vi "Send_TX.vi"(6 "frames (1)":u32=1, 7 "TLS connection":refnum<k5>, 8 "error in (no error)":errorcluster, 9 "status in":T1, 10 "length":i32, 11 "tx":u8[](array[numeric])) -> (0 "error out":errorcluster, 1 "status out":T1)   [LabVIEW 2021, in "CANsub_API.lvlib"]
doc: "API private: sends the first length bytes of the TX buffer with one TCP Write (1000 ms), counts frames written. TCP error ? state = Lost, error 5203. Loop-safe: no allocation, bounded time (except LabVIEW’s TCP Write string)."
uses:
  CANsub_API.lvlib
  Typedefs/CANsub_State.ctl
  common/Typedefs/Bit_Timing.ctl
  common/CANsub_Common.lvlib
  Typedefs/CANsub_Status.ctl
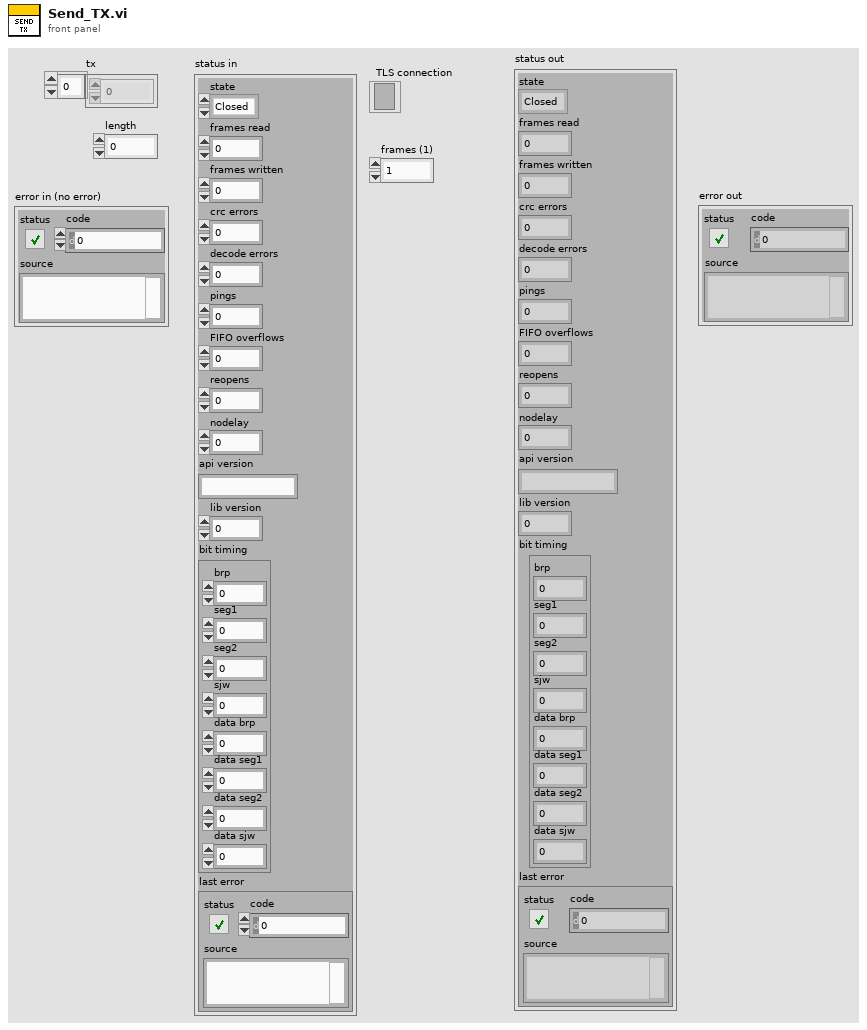
[diagram p1: front panel]
types:
  T1 = typedef "CANsub_API.lvlib/CANsub_Status.ctl" = cluster{"state":T2, "frames read":u32, "frames written":u32, "crc errors":u32, "decode errors":i32, "pings":u32, "FIFO overflows":u32, "reopens":u32, "nodelay":i32, "api version":string, "lib version":u32, "bit timing":T3, "last error":errorcluster}
  T2 = typedef "CANsub_API.lvlib/CANsub_State.ctl" = enum16{"Closed", "Open", "Lost"}
  T3 = typedef "CANsub_Common.lvlib/Bit_Timing.ctl" = cluster{"brp":u16, "seg1":u16, "seg2":u16, "sjw":u16, "data brp":u16, "data seg1":u16, "data seg2":u16, "data sjw":u16}
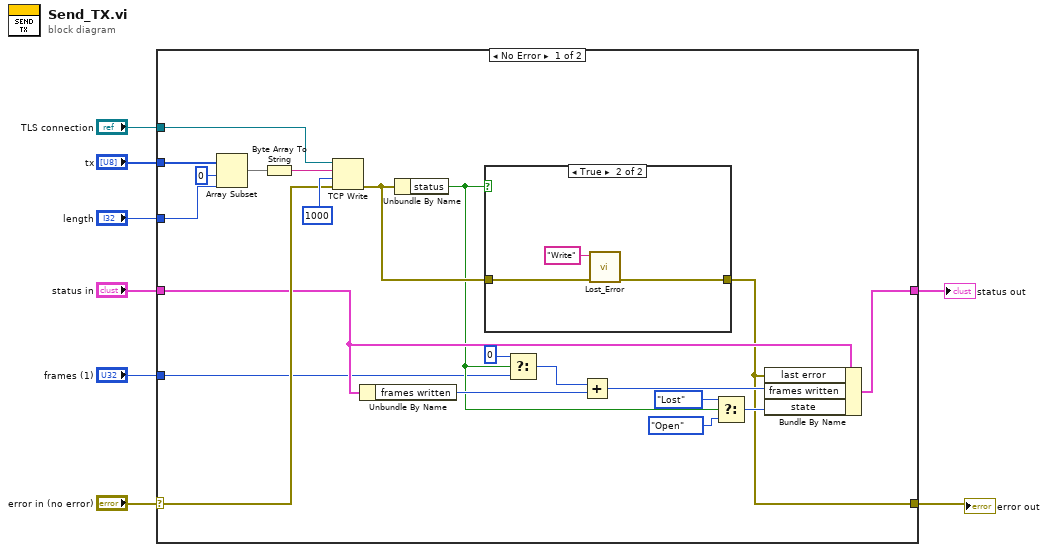
[diagram p0: block diagram]
diagram:
  n1 = case shown="No Error" "error in (no error)" {
    selector: "error in (no error)" -> [w22 w35]
    tunnel: [w10 w35] -> w7
    tunnel: [w19 w34] -> w6
    tunnel: "status in" -> [w20 w34]
    tunnel: "tx" -> [w29 _]
    tunnel: "length" -> [w28 _]
    tunnel: "TLS connection" -> [w24 _]
    tunnel: "frames (1)" -> [w9 _]
    frame No Error {
      n2 = Array Subset(array=w29, index=0, length=w28) -> (w26:u8[])
      n3 = Byte Array To String(unsigned byte array=w26) -> (string=w25:string)
      n4 = TCP Write(connection ID=w24, data in=w25, error in (no error)=w22, 9:1000 ("timeout ms (25000)")) -> (error out=w21:errorcluster)  [unwired: 2 out]
      n5 = Unbundle By Name(w20) -> ("frames written"=w18:u32)
      n6 = Unbundle By Name(w21) -> ("status"=w14:bool)
      n7 = case shown="True" w14 {
        tunnel: w21 -> [w30 w32]
        tunnel: [w30 w31] -> w10
        frame False {
        }
        frame True {
          n8 = call "Lost_Error.vi"("cause"=w32, "operation"="Write") -> ("error out"=w31:errorcluster)  [unwired: 9 in]
        }
      }
      n9 = Select(t=u32 0 ("frames written"), s=w14, f=w9) -> (s? t:f=w16:u32)
      n10 = Add(x=w16, y=w18) -> (x+y=w15:u32)
      n11 = Select(t=CANsub_State."Lost" ("state"), s=w14, f=CANsub_State."Open" ("state")) -> (s? t:f=w11:T2)
      n12 = Bundle By Name(cluster=w20, "last error"=w10, "frames written"=w15, "state"=w11) -> (w19:T1)
    }
    frame Error {
    }
  }
  "status out" <- w6
  "error out" <- w7
